vi "query ACLR Power Value.vi"(8 "error in (no error)":errorcluster, 10 "Measurement Window Mode":T1=enum."MCACpower", 11 "Keysight 9020A in":refnum<class "Keysight 9020A.lvclass">) -> (0 "error out":errorcluster, 2 "Channel Powers":dbl[](array[numeric]), 3 "Keysight 9020A out":refnum<class "Keysight 9020A.lvclass">)   [LabVIEW 2023, in "Spectrum Analyzer.lvlib" / "Keysight 9020A.lvclass"]
uses:
  Keysight 9020A.lvclass
  Keysight 9020A.lvclass/Keysight 9020A.ctl
  TYPE DEFINITION/TYPE Measurement Window Mode.ctl
  Spectrum Analyzer.lvlib
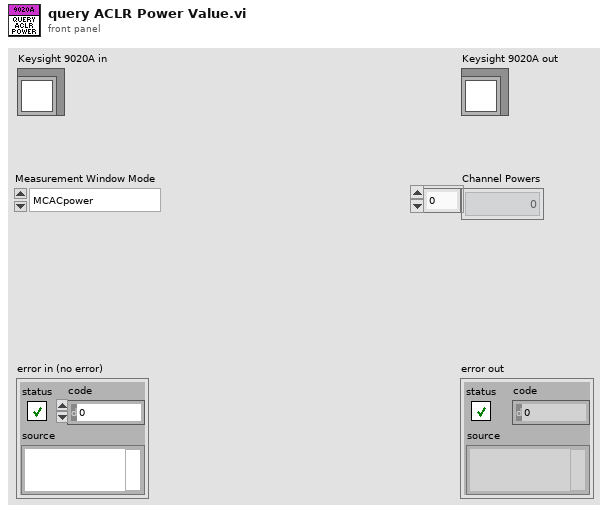
[diagram p1: front panel]
types:
  T1 = typedef "Spectrum Analyzer.lvlib/TYPE Measurement Window Mode.ctl" = enum16{"ACPower", "CPOWer", "MCACpower", "OBANdwidth", "OBWidth", "CN", "CN0"}
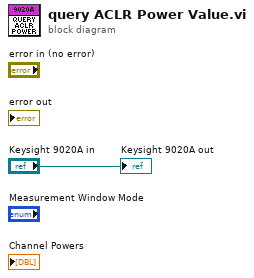
[diagram p0: block diagram]
diagram:
  "Keysight 9020A out" <- "Keysight 9020A in"
